vi "Easy Write XML File.vi"(5 "Encoding (none)":string, 6 "Standalone? (true)":bool=TRUE, 7 "Stylesheet URL (none)":string, 8 "error in (no error)":errorcluster, 9 "Overwrite File? (false)":bool, 10 "LabVIEW Data":variant, 11 "XML File Path":path) -> (0 "error out":errorcluster, 3 "XML File Path (duplicate)":path)   [LabVIEW 2011]
doc: "Converts <B>LabVIEW Data</B> to an XML string and writes it to an XML file with the LabVIEW data names (labels) converted to XML item names and the LabVIEW data values converted to XML item values."
uses:
  <userlib>/_OpenG.lib/lvdata/lvdata.llb/Type Descriptor Enumeration__ogtk.ctl
panel:
  # "JKI EasyXML Toolkit for LabVIEW\nhttp://jki.net/easyxml\nCopyright (C) 2007-2016, JKI <info@jki.net>\nALL RIGHTS RESERVED"
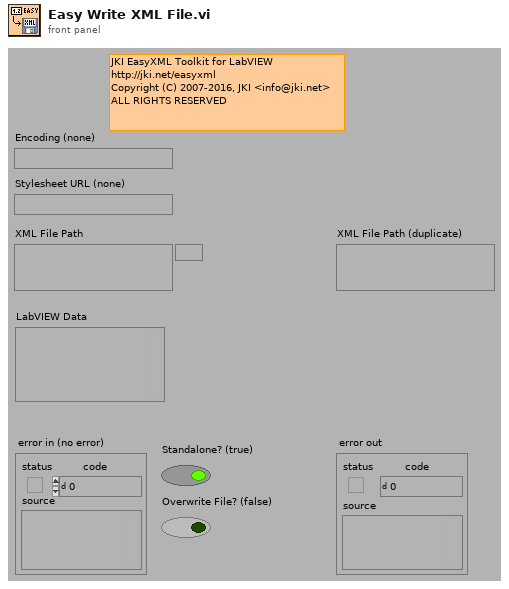
[diagram p1: front panel]
types:
  T1 = enum16{"open", "replace", "create", "open or create", "replace or create", "replace or create with confirmation"}
  T2 = typedef "Type Descriptor Enumeration__ogtk.ctl" = enum8{"<Null>", "I8", "I16", "I32", "I64", "U8", "U16", "U32", "U64", "SGL", "DBL", "EXT", "CSG", "CDB", "CXT", "0x0F", "0x10", "0x11", "0x12", "0x13", "0x14", "Enum U8", "Enum U16", "Enum U32", "Enum U64", "SGL PQ", "DBL PQ", "EXT PQ", "CSG PQ", "CDB PQ", "CXT PQ", "0x1F", "0x20", "Boolean", "0x22", "0x23", "0x24", "0x25", "0x26", "0x27", "0x28", "0x29", "0x2A", "0x2B", "0x2C", "0x2D", "0x2E", "0x2F", "String", "0x31", "Path", "Pict", "0x34", "0x35", "0x36", "DAQ", "0x38", "0x39", "0x3A", "0x3B", "0x3C", "0x3D", "0x3E", "0x3F", "Array", "0x41", "0x42", "0x43", "0x44", "0x45", "0x46", "0x47", "0x48", "0x49", "0x4A", "0x4B", "0x4C", "0x4D", "0x4E", "0x4F", "Cluster", "0x51", "0x52", "Variant", "Waveform", "0x55", "0x56", "0x57", "0x58", "0x59", "0x5A", "0x5B", "0x5C", "0x5D", "0x5E", "0x5F", "0x60", "0x61", "0x62", "0x63", "0x64", "0x65", "0x66", "0x67", "0x68", "0x69", "0x6A", "0x6B", "0x6C", "0x6D", "0x6E", "0x6F", "Refnum"}
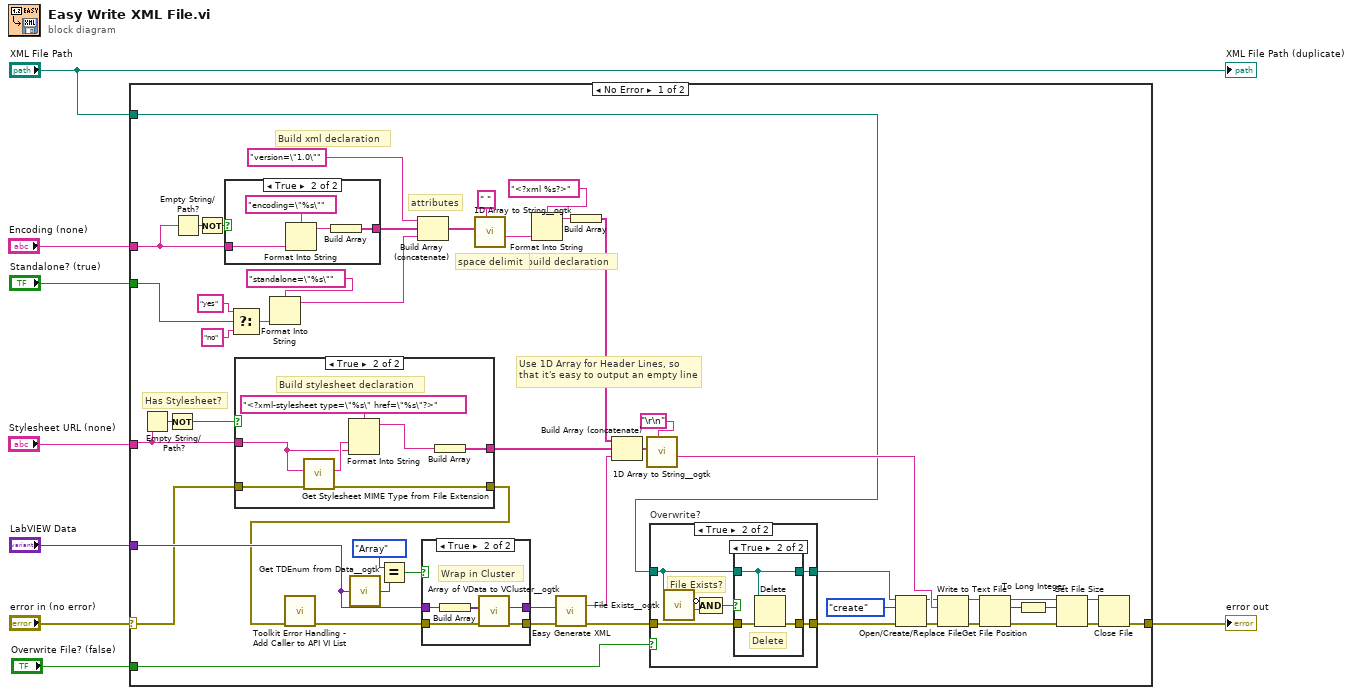
[diagram p0: block diagram]
diagram:
  n1 = case shown="No Error" "error in (no error)" {
    selector: "error in (no error)" -> [w40 w93]
    tunnel: [w47 w93] -> w7
    tunnel: "LabVIEW Data" -> [w54 _]
    tunnel: "XML File Path" -> [w10 _]
    tunnel: "Stylesheet URL (none)" -> [w52 _]
    tunnel: "Encoding (none)" -> [w24 _]
    tunnel: "Standalone? (true)" -> [w50 _]
    tunnel: "Overwrite File? (false)" -> [w11 _]
    frame No Error {
      # "Use 1D Array for Header Lines, so that it's easy to output an empty line"
      # "build declaration"
      # "space delimit"
      # "attributes"
      # "Build xml declaration"
      # "Has Stylesheet?"
      n2 = Empty String/Path?(string/path=w52) -> (empty?=w51:bool)
      n3 = Not(x=w51) -> (.not. x?=w41:bool)
      n4 = Empty String/Path?(string/path=w24) -> (empty?=w23:bool)
      n5 = Not(x=w23) -> (.not. x?=w21:bool)
      n6 = case shown="True" w21 {
        tunnel: w24 -> [_ w76]
        tunnel: [_ w74] -> w22
        frame False {
        }
        frame True {
          n7 = Format Into String(format string="encoding=\"%s\"", w76) -> (resulting string=w75:string)  [unwired: 2 in, 1 out]
          n8 = Build Array(w75) -> (w74:string[])
        }
      }
      n9 = Select(t="yes", s=w50, f="no") -> (s? t:f=w27:string)
      n10 = case shown="True" w41 {
        tunnel: w52 -> [_ w79]
        tunnel: [_ w82] -> w32
        tunnel: [w78 w84] -> w39
        tunnel: w40 -> [w78 w83]
        frame False {
        }
        frame True {
          # "Build stylesheet declaration"
          n11 = call "Get Stylesheet MIME Type from File Extension.vi"("error in"=w83, "Stylesheet URL"=w79) -> ("error out"=w84:errorcluster, "MIME type"=w80:string)  [unwired: 8 in]
          n12 = Format Into String(format string="<?xml-stylesheet type=\"%s\" href=\"%s\"?>", w80, w79) -> (resulting string=w81:string)  [unwired: 2 in, 1 out]
          n13 = Build Array(w81) -> (w82:string[])
        }
      }
      n14 = Format Into String(format string="standalone=\"%s\"", w27) -> (resulting string=w25:string)  [unwired: 2 in, 1 out]
      n15 = call "Toolkit Error Handling - Add Caller to API VI List.vi"("error in"=w39) -> ("error out"=w53:errorcluster)  [unwired: 10 in]
      n16 = call <userlib>:"Get TDEnum from Data__ogtk.vi"("Data"=w54) -> ("Type Descriptor Enumeration"=w59:T2)  [unwired: 4 in]
      n17 = Equal?(x=Type_Descriptor_Enumeration__ogtk."Array" ("Type Descriptor Enumeration"), y=w59) -> (x = y?=w57:bool)
      n18 = Build Array (concatenate)("version=\"1.0\"", w22, w25) -> (w37:string[])
      n19 = case shown="True" w57 {
        tunnel: w53 -> [w87 w91]
        tunnel: [w87 w90] -> w56
        tunnel: w54 -> [w86 w89]
        tunnel: [w86 w88] -> w55
        frame False {
        }
        frame True {
          # "Wrap in Cluster"
          n20 = Build Array(w89) -> (w92:variant[])
          n21 = call <userlib>:"Array of VData to VCluster__ogtk.vi"("error in (no error)"=w91, "Array"=w92) -> ("error out"=w90:errorcluster, "VCluster"=w88:variant)  [unwired: 8 in]
        }
      }
      n22 = call <userlib>:"1D Array to String__ogtk.vi"("delimiter (Tab)"=" ", "Array of Strings"=w37) -> ("delimited string"=w35:string)  [unwired: 9 in]
      n23 = Format Into String(format string="<?xml %s?>", w35) -> (resulting string=w33:string)  [unwired: 2 in, 1 out]
      n24 = call "Easy Generate XML.vi"("error in (no error)"=w56, "LabVIEW Data"=w55) -> ("error out"=w13:errorcluster, "XML String"=w30:string)  [unwired: 8 in]
      n25 = Build Array(w33) -> (w18:string[])
      n26 = Build Array (concatenate)(w18, w32, w30) -> (w31:string[])
      n27 = call <userlib>:"1D Array to String__ogtk.vi"("delimiter (Tab)"="\r\n", "Array of Strings"=w31) -> ("delimited string"=w29:string)  [unwired: 9 in]
      n28 = case "Overwrite?" shown="True" w11 {
        tunnel: [w61 w62] -> w12
        tunnel: w13 -> [w61 w65]
        tunnel: w10 -> [w60 w64]
        tunnel: [w60 w63] -> w9
        frame False {
        }
        frame True {
          # "File Exists?"
          n29 = call <userlib>:"File Exists__ogtk.vi"("file path"=w64) -> ("is directory"=w68:bool, "exists"=w67:bool)  [unwired: 6 in]
          n30 = Compound Arithmetic op=AND(invert w68, w67) -> (w66:bool)
          n31 = case shown="True" w66 {
            tunnel: w65 -> [w69 w73]
            tunnel: w64 -> [w70 w72]
            tunnel: [w70 w72] -> w63
            tunnel: [w69 w71] -> w62
            frame False {
            }
            frame True {
              # "Delete"
              n32 = Delete(path (use dialog)=w72, error in=w73) -> (error out=w71:errorcluster)  [unwired: 3 in, 2 out]
            }
          }
        }
      }
      n33 = Open/Create/Replace File(file path (use dialog)=w9, error in=w12, operation (0:open)=T1."create") -> (refnum out=w19:refnum<file>, error out=w20:errorcluster)  [unwired: 3 in, 1 out]
      n34 = Write to Text File(file (use dialog)=w19, text=w29, error in=w20) -> (refnum out=w16:refnum<file>, error out=w15:errorcluster)  [unwired: 1 in, 1 out]
      n35 = Get File Position(4:w15, 7:w16) -> (0:w46:errorcluster, 2:w14:i64, 3:w45:refnum<file>)
      n36 = To Long Integer(number=w14) -> (32bit integer=w42:i32)
      n37 = Set File Size(4:w46, 6:w42, 7:w45) -> (0:w43:errorcluster, 3:w44:refnum<file>)
      n38 = Close File(refnum=w44, error in=w43) -> (error out=w47:errorcluster)  [unwired: 1 out]
    }
    frame Error {
    }
  }
  "error out" <- w7
  "XML File Path (duplicate)" <- "XML File Path"
